vi "Debug Screen.vi"() -> ()   [LabVIEW 2013]
uses:
  Host/FGs/FPGA_Reference.ctl
  Common/CL Configuration.ctl
  Common/CL Signal Mapping.ctl
  <vilib>/rvi/interface/nirviReadWriteControl/nirviReadWriteControl.xnode
  NiFpgaLv.dll
  <vilib>/Utility/error.llb/Error Cluster From Error Code.vi
  <vilib>/rvi/errors/niLvFpgaAdjustHostInterfaceError.vi
  <vilib>/rvi/interface/nirviMethod/nirviMethod.xnode
  <vilib>/FPGAPlugInAG/PCIe-1473R/niLvFpga_ReadFifo_PCIe-1473R.vi
  <vilib>/rvi/errors/niLvFpgaMergeErrorWithErrorCode.vi
  FPGA Bitfiles/8-Tap8-bitCamera_FPGATarget_8-Tap8-bit_Serial_Server.lvbitx
panel:
  out "Y Resolution":u16
  out "X Resolution":u16
  out "Accumulated":T1(array[cluster])
  out "Sector pixel locations":T2(array[cluster])
  out "Analysis Ticks":u32
  out "Acq Control.Initialize":bool
  out "Acq Control.Ignore DVAL 2":bool
  out "Acq Control.Cancel Acq":bool
  out "Acq Control.Acquire 2":bool
  out "Acq Control.Frames To Acq":u32
  out "Acq Control.Line Scan Height":u32
  out "Acq Status.Initialized":bool
  out "Acq Status.DMA Write Timeout":bool
  out "Acq Status.Lines Per Frame":u32
  out "Acq Status.Frames Acq'd":u32
  out "Acq Status.Clocks Per Line":u32
  out "Acq Status.Acq In Progress":bool
  out "# of Frames to Average":u8
  out "CL Config.Signal Mapping":T3
  out "Acq Control.Acquire":bool
  out "CL Config.Configuration":T4
  out "Acq Control.Ignore DVAL":bool
  out "CL Config.Line Scan":bool
  out "CL Config.Spare Active High":bool
  out "CL Config.DVAL Active High":bool
  out "CL Config.LVAL Active High":bool
  out "CL Config.FVAL Active High":bool
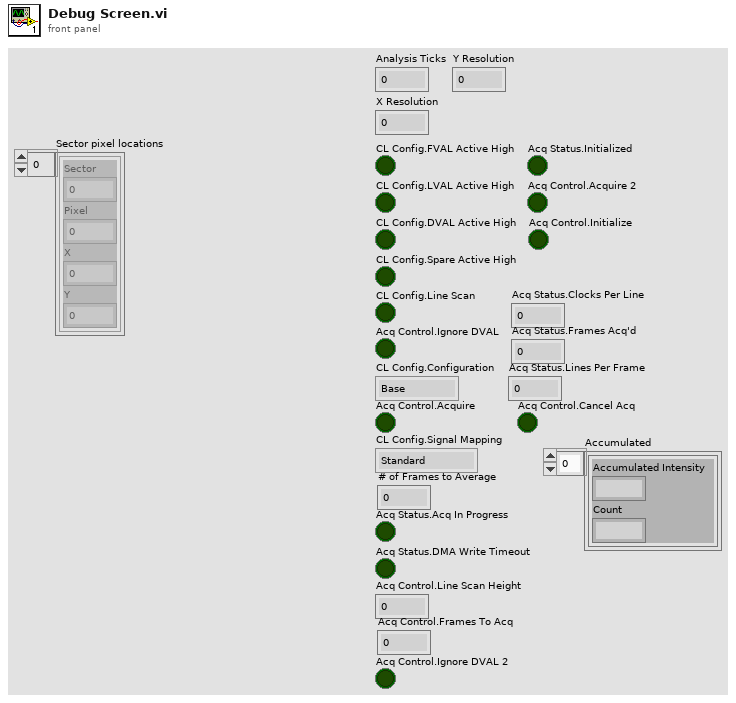
[diagram p1: front panel]
types:
  T1 = cluster{"Accumulated Intensity":fxp<+,20,20>, "Count":fxp<+,12,12>}[]
  T2 = cluster{"Sector":dbl, "Pixel":dbl, "X":dbl, "Y":dbl}[]
  T3 = typedef "CL Signal Mapping.ctl" = enum8{"Standard", "Basler 10-tap", "Vosskühler 10-tap"}
  T4 = typedef "CL Configuration.ctl" = enum8{"Base", "Medium", "Full"}
  T5 = typedef "FPGA_Reference.ctl" = refnum<k20>
  T6 = cluster{"Sector":dbl, "Pixel":dbl, "X":dbl, "Y":dbl}
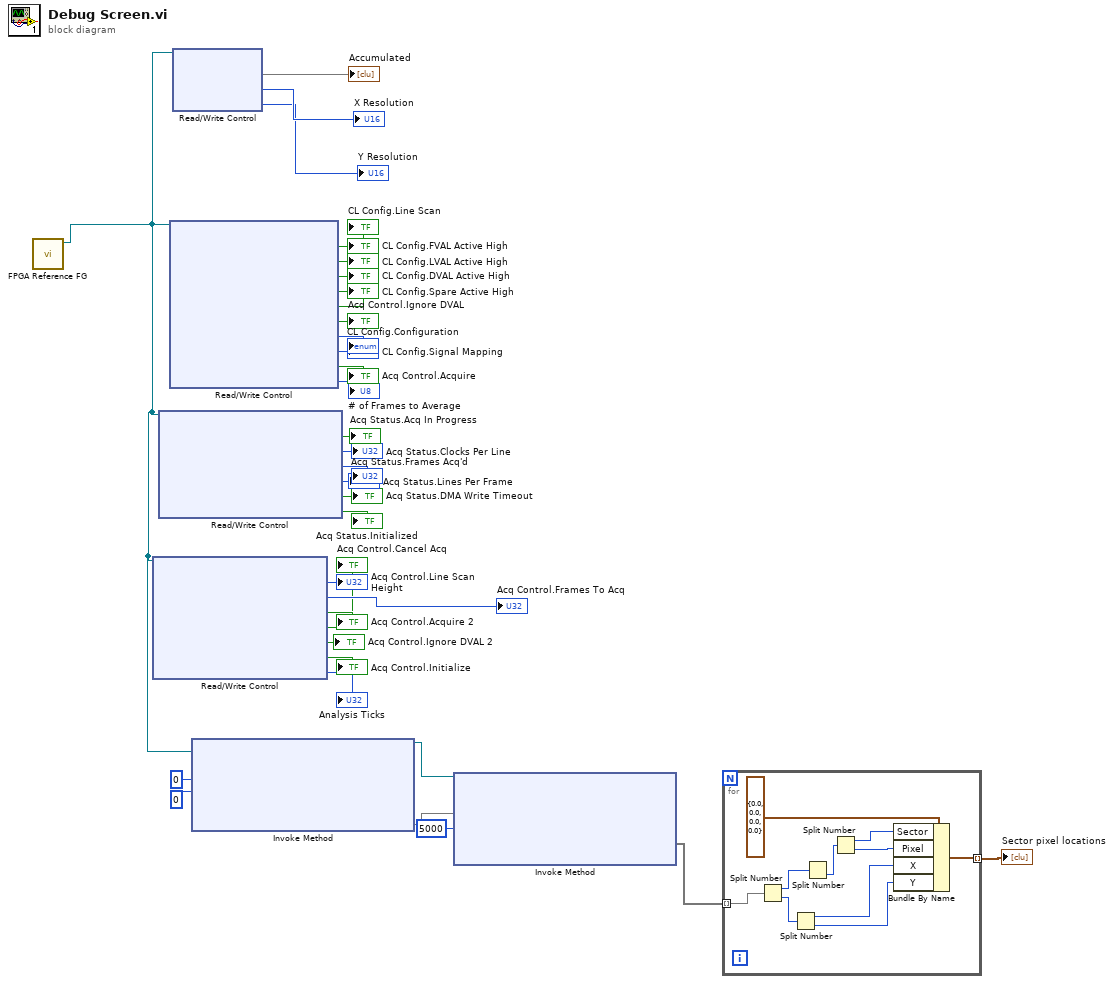
[diagram p0: block diagram]
diagram:
  n1 = call "FPGA Reference FG.vi"() -> ("FPGA VI Reference Out"=w4:T5)  [unwired: 11 in]
  n2 = xnode "Read/Write Control"("FPGA VI Reference In"=w4) -> ("Acq Control.Line Scan Height"=→"Acq Control.Line Scan Height":u32, "Acq Control.Frames To Acq"=→"Acq Control.Frames To Acq":u32, "Acq Control.Acquire"=→"Acq Control.Acquire 2":bool, "Acq Control.Cancel Acq"=→"Acq Control.Cancel Acq":bool, "Acq Control.Ignore DVAL"=→"Acq Control.Ignore DVAL 2":bool, "Acq Control.Initialize"=→"Acq Control.Initialize":bool, "Analysis Ticks"=→"Analysis Ticks":u32)  [unwired: 1 in, 2 out]
  n3 = xnode "Read/Write Control"("FPGA VI Reference In"=w4) -> ("Acq Status.Acq In Progress"=→"Acq Status.Acq In Progress":bool, "Acq Status.Clocks Per Line"=→"Acq Status.Clocks Per Line":u32, "Acq Status.Frames Acq'd"=→"Acq Status.Frames Acq'd":u32, "Acq Status.Lines Per Frame"=→"Acq Status.Lines Per Frame":u32, "Acq Status.DMA Write Timeout"=→"Acq Status.DMA Write Timeout":bool, "Acq Status.Initialized"=→"Acq Status.Initialized":bool)  [unwired: 1 in, 2 out]
  n4 = xnode "Read/Write Control"("FPGA VI Reference In"=w4) -> ("CL Config.FVAL Active High"=→"CL Config.FVAL Active High":bool, "CL Config.LVAL Active High"=→"CL Config.LVAL Active High":bool, "CL Config.DVAL Active High"=→"CL Config.DVAL Active High":bool, "CL Config.Spare Active High"=→"CL Config.Spare Active High":bool, "CL Config.Line Scan"=→"CL Config.Line Scan":bool, "Acq Control.Ignore DVAL"=→"Acq Control.Ignore DVAL":bool, "CL Config.Configuration"=→"CL Config.Configuration":T4, "CL Config.Signal Mapping"=→"CL Config.Signal Mapping":T3, "Acq Control.Acquire"=→"Acq Control.Acquire":bool, "# of Frames to Average"=→"# of Frames to Average":u8)  [unwired: 1 in, 2 out]
  n5 = xnode "Read/Write Control"("FPGA VI Reference In"=w4) -> ("Accumulated"=→"Accumulated", "X Resolution"=→"X Resolution":u16, "Y Resolution"=→"Y Resolution":u16)  [unwired: 1 in, 2 out]
  n6 = xnode "Invoke Method"("FPGA VI Reference In"=w4, "Number of Elements"=u32 0, "Timeout (ms)"=0) -> ("FPGA VI Reference Out"=w5:T5, "Elements Remaining"=w8)  [unwired: 1 in, 2 out]
  n7 = xnode "Invoke Method"("FPGA VI Reference In"=w5, "Number of Elements"=w8, "Timeout (ms)"=5000) -> ("Data"=w7:void[])  [unwired: 1 in, 3 out]
  n8 = for {
    tunnel: w7 -> [w44] mode=indexing
    tunnel: [w38] -> w9 mode=indexing
    n9 = Split Number(x=w44) -> (hi(x)=w43:u16, lo(x)=w42:u16)
    n10 = Split Number(x=w42) -> (hi(x)=w40:u8, lo(x)=w39:u8)
    n11 = Split Number(x=w43) -> (lo(x)=w37:u8)  [unwired: 1 out]
    n12 = Split Number(x=w37) -> (hi(x)=w36:u8, lo(x)=w35:u8)
    n13 = Bundle By Name(cluster=T6 {"Sector"=0.0, "Pixel"=0.0, "X"=0.0, "Y"=0.0} ("Cluster"), "Sector"=w36, "Pixel"=w35, "X"=w40, "Y"=w39) -> (w38:T6)
  }
  "Sector pixel locations" <- w9
